vi "XNET CAN to Header Cluster.vi"(10 "Interface Mode":T4, 11 "XNET CAN frame":T1 {"payload" format="%x"; "timestamp" format="%<%.7X\n%x>T"; "type" items=["CAN Data"=0, "CAN Remote"=1, "CAN Bus Error"=2, "CAN 2.0 Data"=8, "CAN FD Data"=16, "CAN FD+BRS Data"=24, "J1939 Data"=192, "Delay"=224, "Log Trigger"=225, "Start Trigger"=226]; "identifier" format="%x"}) -> (1 "Total Length":i32, 2 "TAI Time (ns)":i64, 3 "CAN Header out":T3 {"CANID and Flags" format="%.0x"; "FD Flags" format="%.0x"}, 5 "Unsupported":bool)   [LabVIEW 2021, in "XNET CAN RW.lvclass"]
uses:
  XNET CAN RW.lvclass
  <vilib>/CIF Foundation/CIF CAN RW Core/typedef/CAN Interface Mode.ctl
  <vilib>/CIF Foundation/CIF PCAP Parse and Build/Typedef/Format Specific/Socket CAN Header.ctl
  <vilib>/xnet/xnet.llb/XNET Frame CAN.ctl
  <vilib>/xnet/xnet.llb/XNET Frame Type CAN.ctl
  XNET CAN RW.lvclass/XNET CAN RW.ctl
  <vilib>/CIF Foundation/CIF Utilities/Time/Time_CIF_U.lvlib
  <vilib>/CIF Foundation/CIF PCAP Parse and Build/pcap_Parse_Build_CIF.lvclass
  <vilib>/CIF Foundation/CIF CAN RW Core/CAN_RW_CORE.lvclass
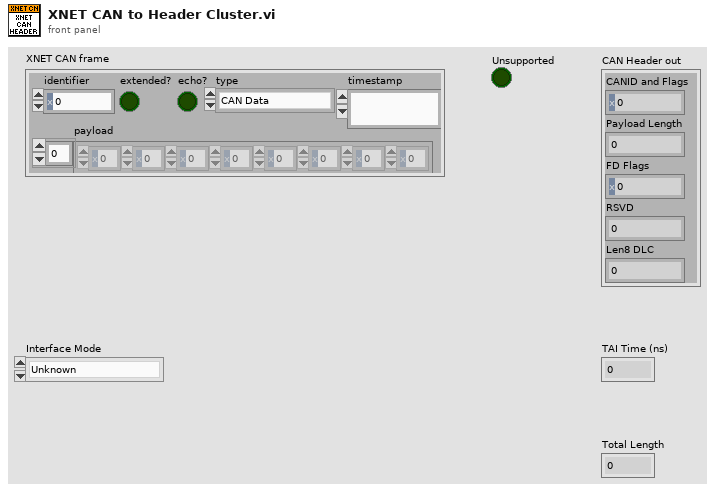
[diagram p1: front panel]
types:
  T1 = typedef "XNET Frame CAN.ctl" = cluster{"timestamp":timestamp, "payload":u8[], "identifier":u32, "type":T2, "extended?":bool, "echo?":bool}
  T2 = typedef "XNET Frame Type CAN.ctl" = u8
  T3 = typedef "pcap_Parse_Build_CIF.lvclass/Socket CAN Header.ctl" = cluster{"CANID and Flags":u32, "Payload Length":u8, "FD Flags":u8, "RSVD":u8, "Len8 DLC":u8}
  T4 = typedef "CAN_RW_CORE.lvclass/CAN Interface Mode.ctl" = enum16{"Unknown", "CAN 2.0", "CAN FD", "CAN FD BRS"}
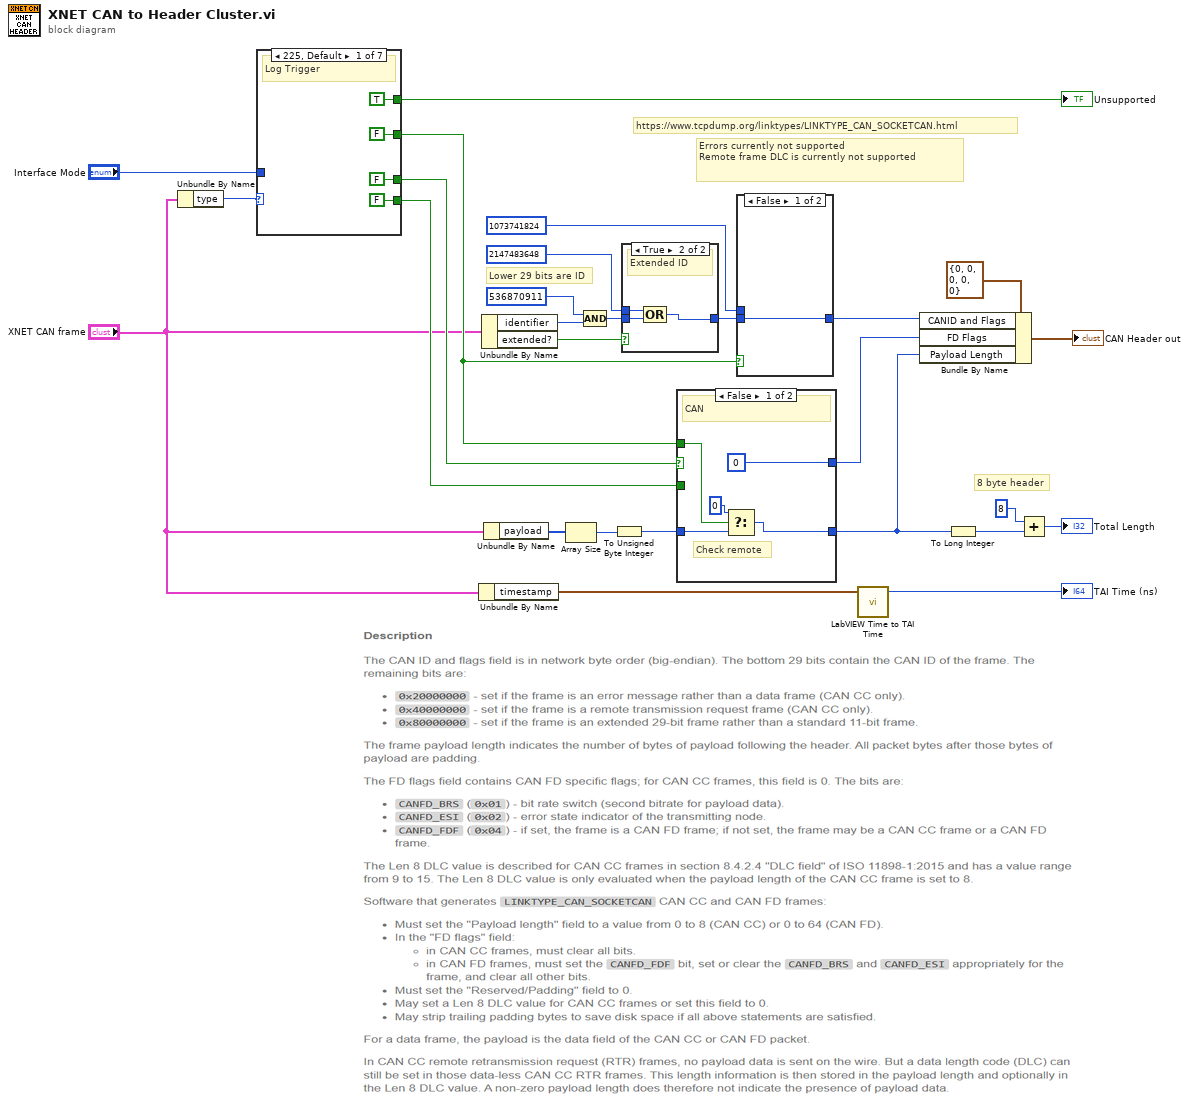
[diagram p0: block diagram]
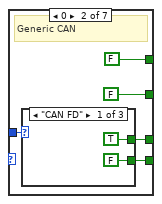
[diagram p2: hidden frame]
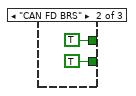
[diagram p3: hidden frame]
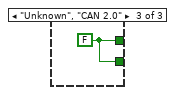
[diagram p4: hidden frame]
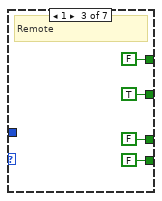
[diagram p5: hidden frame]
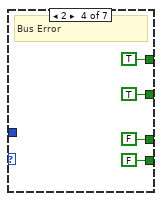
[diagram p6: hidden frame]
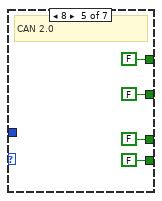
[diagram p7: hidden frame]
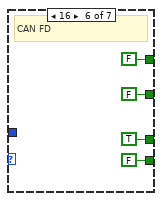
[diagram p8: hidden frame]
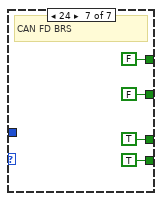
[diagram p9: hidden frame]
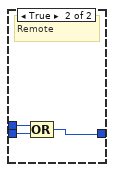
[diagram p10: hidden frame]
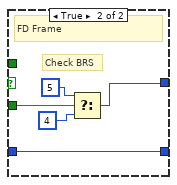
[diagram p12: hidden frame]
diagram:
  # "8 byte header"
  # "Errors currently not supported\nRemote frame DLC is currently not supported"
  # "Lower 29 bits are ID"
  # "https://www.tcpdump.org/linktypes/LINKTYPE_CAN_SOCKETCAN.html"
  n1 = Unbundle By Name("XNET CAN frame") -> ("type"=w16:T2)
  n2 = case shown="225, Default" w16 {
    tunnel: "Interface Mode" -> [_ w35 _ _ _ _ _]
    tunnel: [FALSE FALSE TRUE TRUE FALSE FALSE FALSE] -> w13
    tunnel: [FALSE w34 FALSE FALSE FALSE TRUE TRUE] -> w10
    tunnel: [FALSE w33 FALSE FALSE FALSE FALSE TRUE] -> w11
    tunnel: [TRUE FALSE FALSE TRUE FALSE FALSE FALSE] -> w14
    frame 225, Default {
      # "Log Trigger"
    }
    frame 0 {
      # "Generic CAN"
      n3 = case shown="\"CAN FD\"" w35 {
        tunnel: [TRUE TRUE w41] -> w34
        tunnel: [FALSE TRUE w41] -> w33
        frame "CAN FD" {
        }
        frame "CAN FD BRS" {
        }
        frame "Unknown", "CAN 2.0" {
          w41 = FALSE
        }
      }
    }
    frame 1 {
      # "Remote"
    }
    frame 2 {
      # "Bus Error"
    }
    frame 8 {
      # "CAN 2.0"
    }
    frame 16 {
      # "CAN FD"
    }
    frame 24 {
      # "CAN FD BRS"
    }
  }
  "Unsupported" <- w14
  n4 = Unbundle By Name("XNET CAN frame") -> ("timestamp"=w9:timestamp)
  n5 = Unbundle By Name("XNET CAN frame") -> ("identifier"=w18:u32, "extended?"=w17:bool)
  n6 = Unbundle By Name("XNET CAN frame") -> ("payload"=w20:u8[])
  n7 = Array Size(array=w20) -> (size(s)=w19:i32)
  n8 = Compound Arithmetic op=AND(u32 536870911 ("number"), w18) -> (w26:u32)
  n9 = To Unsigned Byte Integer(number=w19) -> (unsigned 8bit integer=w12:u8)
  n10 = case shown="True" w17 {
    tunnel: w26 -> [w62 w65]
    tunnel: u32 2147483648 -> [_ w64]
    tunnel: [w62 w63] -> w24
    frame False {
    }
    frame True {
      # "Extended ID"
      n11 = Compound Arithmetic op=OR(w64, w65) -> (w63:u32)
    }
  }
  n12 = case shown="False" w10 {
    tunnel: w11 -> [_ w74]
    tunnel: [u8 0 w71] -> w21
    tunnel: w12 -> [w69 w75]
    tunnel: [w66 w75] -> w7
    tunnel: w13 -> [w68 _]
    frame False {
      # "Check remote"
      # "CAN"
      n13 = Select(t=u8 0, s=w68, f=w69) -> (s? t:f=w66:u8)
    }
    frame True {
      # "Check BRS"
      # "FD Frame"
      n14 = Select(t=u8 5, s=w74, f=u8 4) -> (s? t:f=w71:u8)
    }
  }
  n15 = case shown="False" w13 {
    tunnel: w24 -> [w76 w79]
    tunnel: [w76 w78] -> w22
    tunnel: u32 1073741824 -> [_ w77]
    frame False {
    }
    frame True {
      # "Remote"
      n16 = Compound Arithmetic op=OR(w77, w79) -> (w78:u32)
    }
  }
  n17 = call <vilib>:"LabVIEW Time to TAI Time.vi"("LabVIEW Time (s)"=w9) -> ("TAI Time (ns)"=→"TAI Time (ns)":i64)  [unwired: 4 in]
  n18 = Bundle By Name(cluster=T3 {"CANID and Flags"=0, "Payload Length"=0, "FD Flags"=0, "RSVD"=0, "Len8 DLC"=0} ("CAN Header out 2"), "CANID and Flags"=w22, "FD Flags"=w21, "Payload Length"=w7) -> (→"CAN Header out":T3)
  n19 = To Long Integer(number=w7) -> (32bit integer=w4:i32)
  n20 = Add(x=8, y=w4) -> (x+y=→"Total Length":i32)
